vi "Acquisition.vi"(7 "CSM Name":string="CSM-Module") -> ()   [LabVIEW 2026, in "UI-温度控制.lvlib" / "Acquisition.lvlib"]
uses:
  Acquisition.lvlib
  Supports/Acquiring States.ctl
  Supports/Device Info.ctl
  Data ColndSave/Supports/Time and Data.ctl
  7c1bd55a-2ec8-456f-bad7-7e130b55c93f.vi
  2e6eb7ec-e133-45c6-ba3a-bbdf519762d0.vi
  817e4cca-a27d-44f6-a578-b7f1dff5f736.vi
  e4661991-72f6-45df-8df2-cd331cd0573d.vi
  d2ac0b8d-a34d-4c44-96e2-60a2cc9ef1dc.vi
  396d3fb3-9d86-4935-bc9b-05414301d3b2.vi
  e2432089-641f-414f-ac69-b6d04279e506.vi
  144ef8d5-f062-4612-a884-90947adc4c96.vi
  <userlib>/_NEVSTOP/Communicable State Machine(CSM)/AdvanceAPI/CSM - Revert Arguments-Safe String.vi
  <userlib>/_NEVSTOP/Communicable State Machine(CSM)/_Shared/Trim Single-line Text.vi
  <userlib>/_NEVSTOP/Communicable State Machine(CSM)/AdvanceAPI/CSM - Make String Arguments Safe.vi
  <userlib>/_NEVSTOP/Communicable State Machine(CSM)/AdvanceAPI/CSM - Break Down Multiple States String.vi
  <userlib>/_NEVSTOP/Communicable State Machine(CSM)/AdvanceAPI/CSM - Compact Multiple States.vi
  <userlib>/_NEVSTOP/Communicable State Machine(CSM)/AdvanceAPI/CSM - Keywords.vi
  <userlib>/_NEVSTOP/Communicable State Machine(CSM)/addons/API-String-Arugments-Support/_Support/Convert API String Arguments to Data(variant).vi
  <userlib>/_NEVSTOP/Communicable State Machine(CSM)/addons/MassData-Parameter/_support/FGV-MassData(lvlibp).vi
  <userlib>/_NEVSTOP/Communicable State Machine(CSM)/Communicable State Machine.lvlib
  <userlib>/_NEVSTOP/Communicable State Machine(CSM)/addons/Loop-Support/CSM Loop Support.lvlib
  Data ColndSave/Data Collection and Save.lvlib
panel:
  out "Error Occurred":errorcluster
  out "State History":string
  in  "Exit":bool
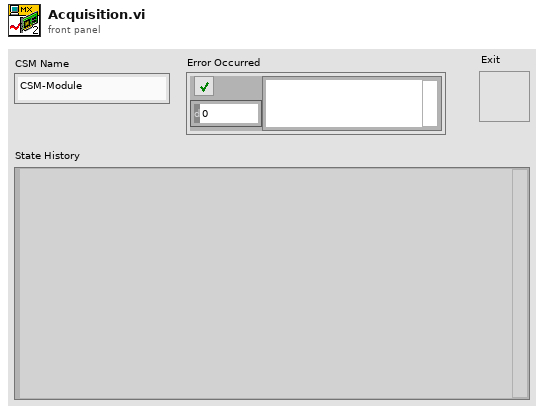
[diagram p1: front panel]
types:
  T1 = enum32{"Invalid", "Standard", "Closed", "Hidden", "Minimized", "Maximized"}
  T2 = enum32{"invalid app kind", "Development System", "Run Time System", "Student Edition", "Embedded LabVIEW", "Evaluation", "Custom"}
  T3 = typedef "UI-温度控制.lvlib/Acquisition.lvlib/Acquiring States.ctl" = enum16{"Idle", "Acquiring", "Error"}
  T4 = typedef "Data Collection and Save.lvlib/Time and Data.ctl" = cluster{"采集时间":timestamp, "Data":dbl[]}
  T5 = typedef "Communicable State Machine.lvlib/_CSM_Response Source Message.ctl" = cluster{"‘State":string, "’Arguments":string, "’Error":errorcluster}
  T6 = cluster{"Current VI Reference":refnum<vi>, "Close Panel on Exit?":bool}
  T7 = typedef "UI-温度控制.lvlib/Device Info.ctl" = cluster{"基本信息":cluster{"USB Port":refnum<visa-resource-name>, "采集间隔(s)":dbl}, "设备信息":cluster{"设备型号":string, "双通道设备？":bool}, "开关":cluster{"开关 1":bool, "开关 2":bool, "Fast Mode":bool}, "Control Temp":cluster{"Control Temp 1":dbl, "Control Temp 2":dbl}}
  T8 = cluster{"Core":cluster{"Current VI Reference":refnum<vi>, "Close Panel on Exit?":bool}, "State":T3, "Device Info":T7, "采集时间":timestamp}
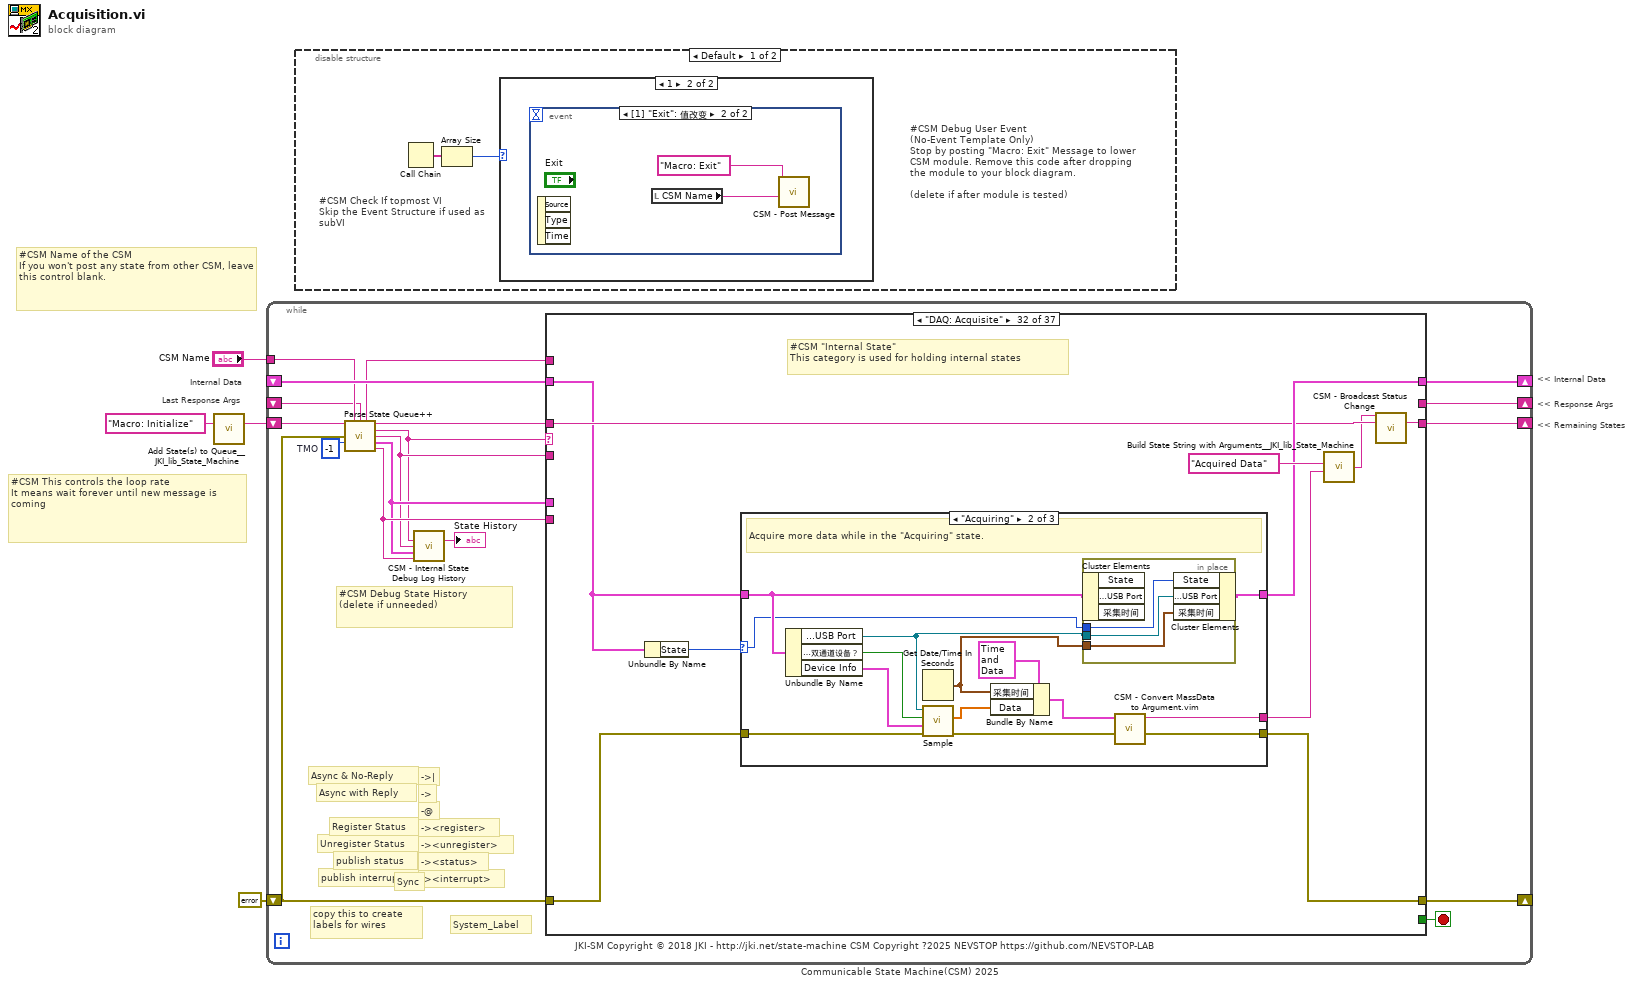
[diagram p0: block diagram]
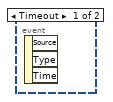
[diagram p3: hidden frame]
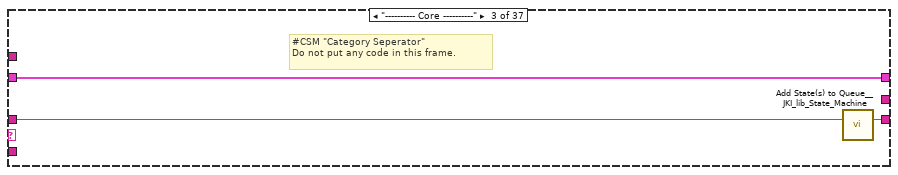
[diagram p7: hidden frame]
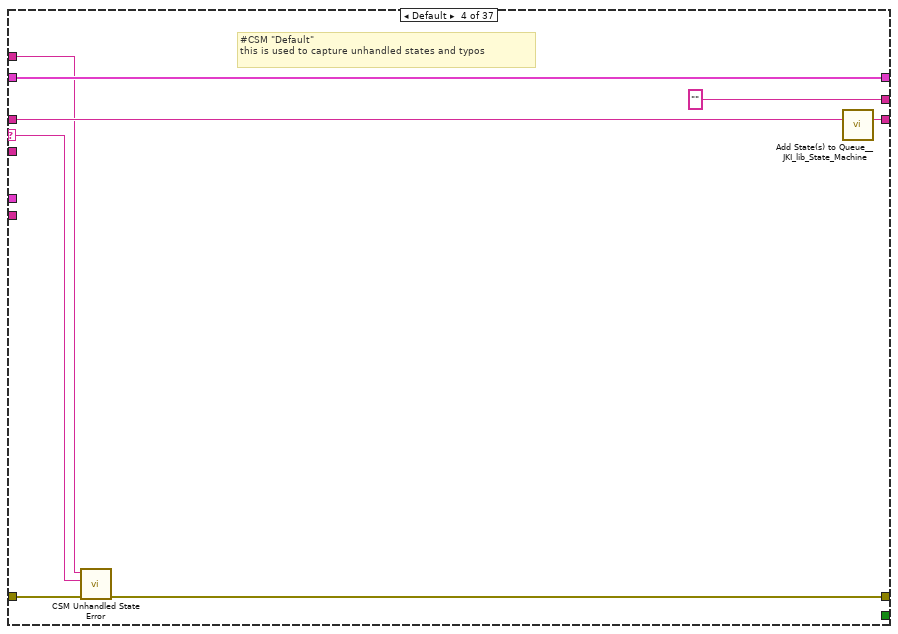
[diagram p8: hidden frame]
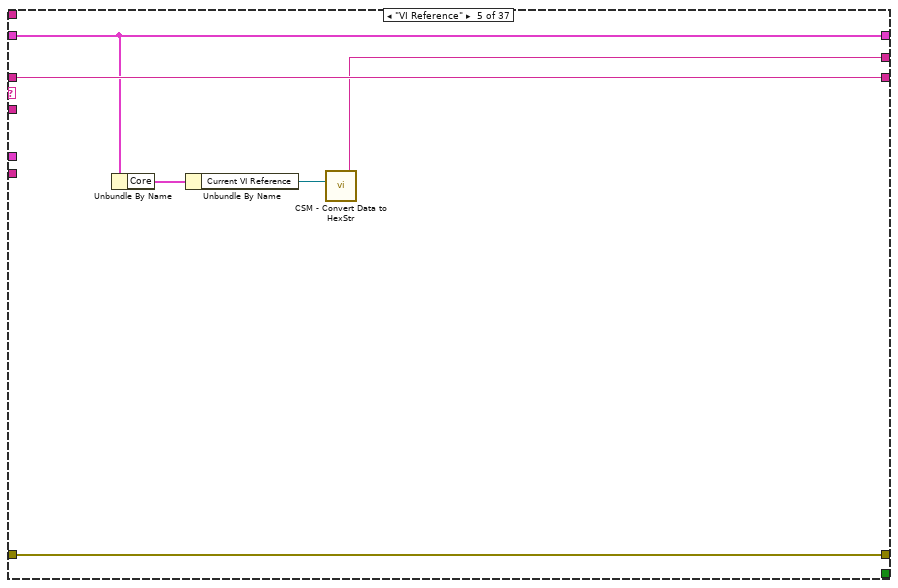
[diagram p9: hidden frame]
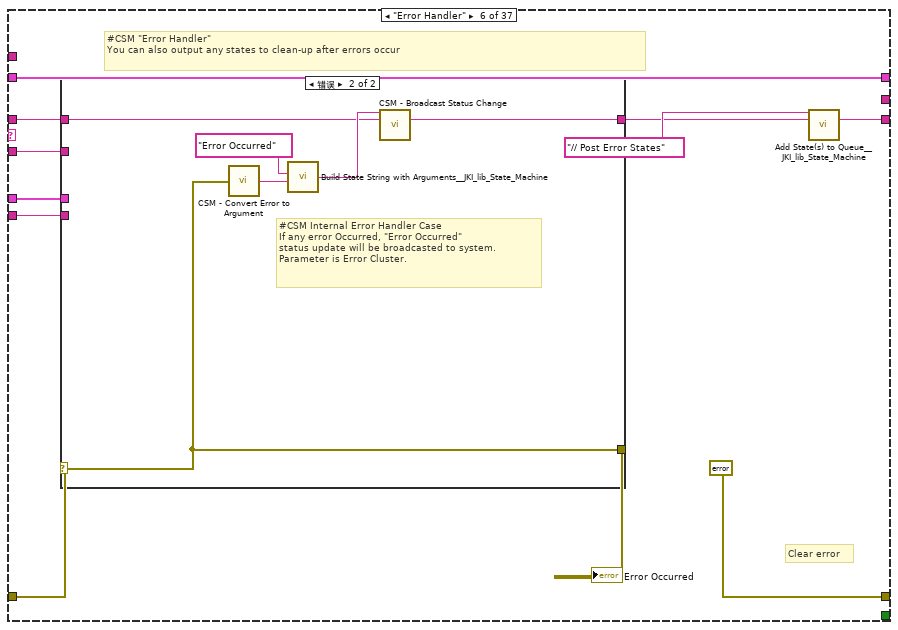
[diagram p10: hidden frame]
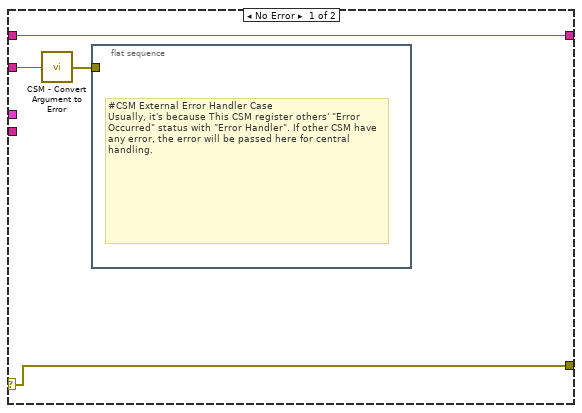
[diagram p11: hidden frame]
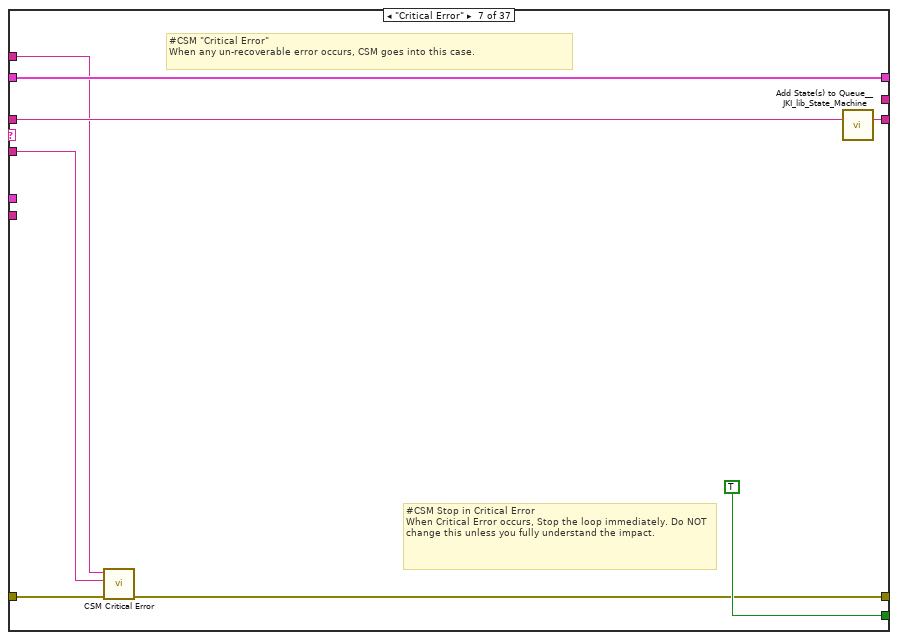
[diagram p12: hidden frame]
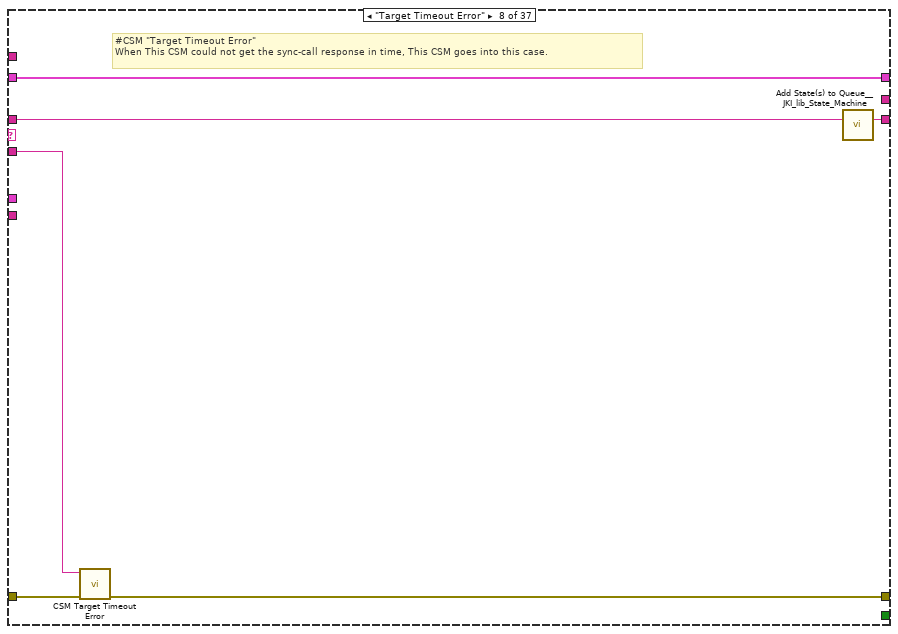
[diagram p13: hidden frame]
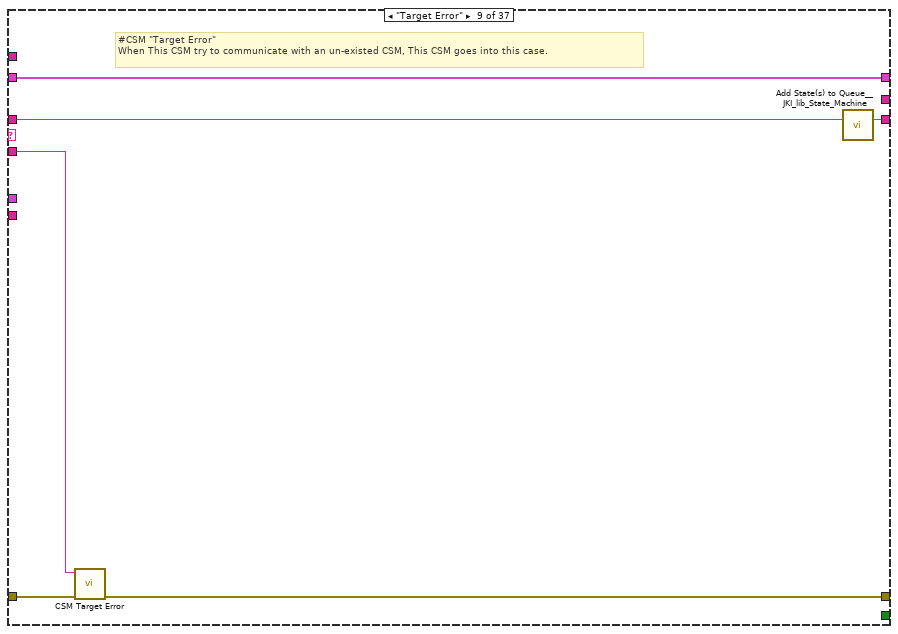
[diagram p14: hidden frame]
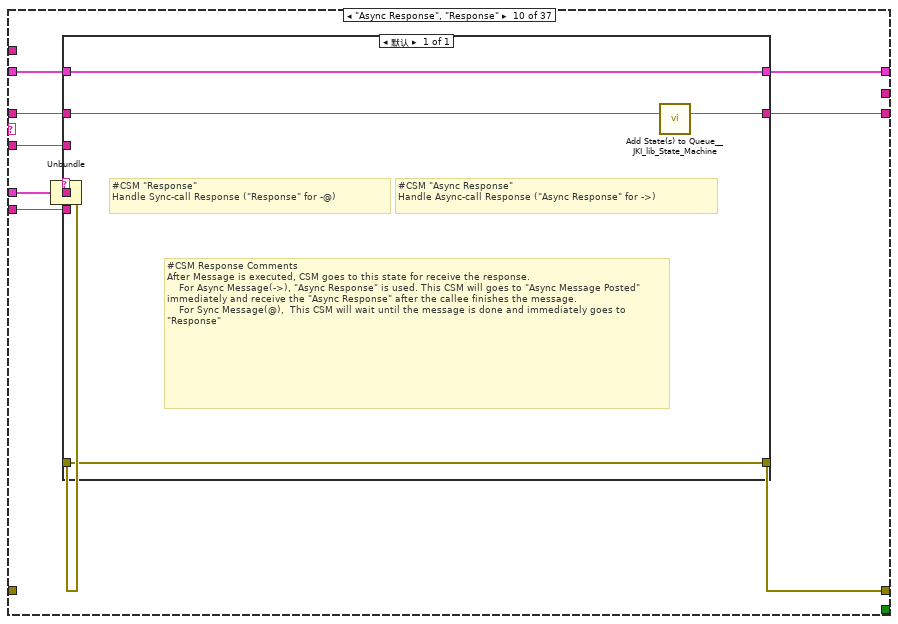
[diagram p15: hidden frame]
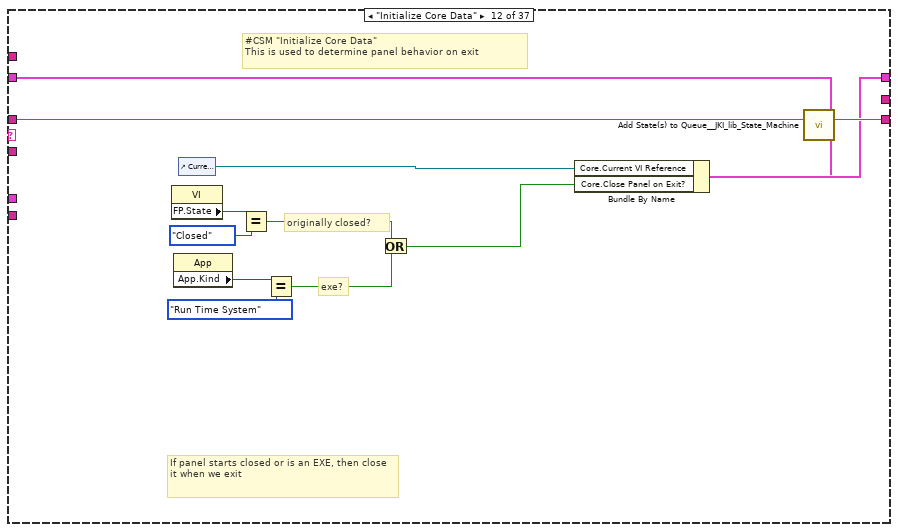
[diagram p17: hidden frame]
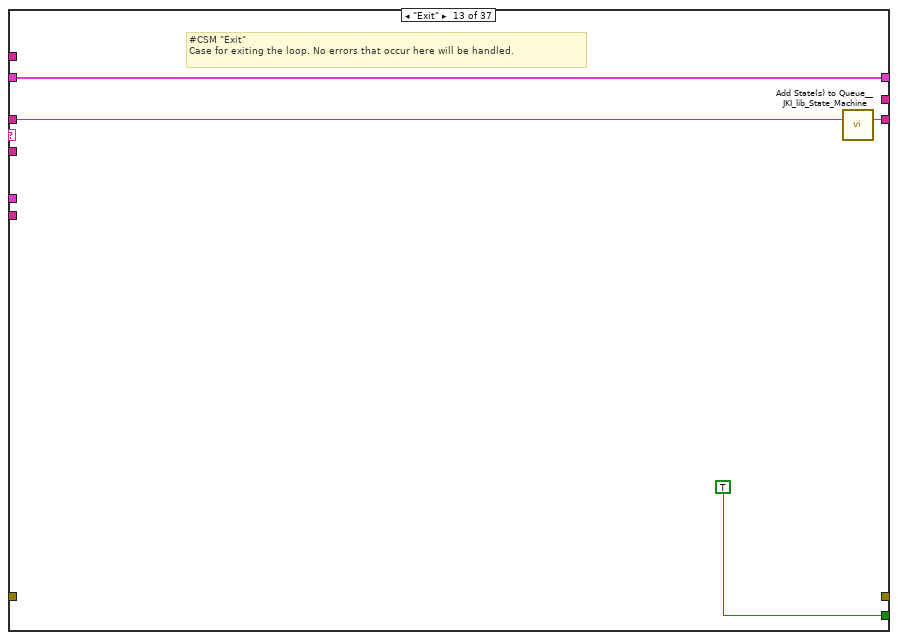
[diagram p18: hidden frame]
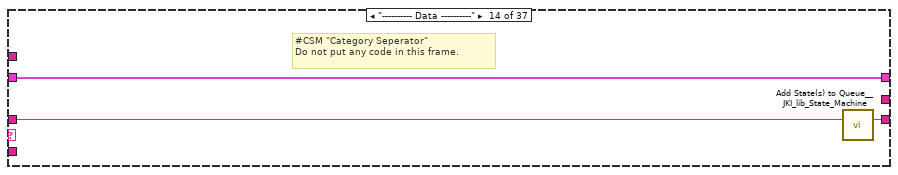
[diagram p19: hidden frame]
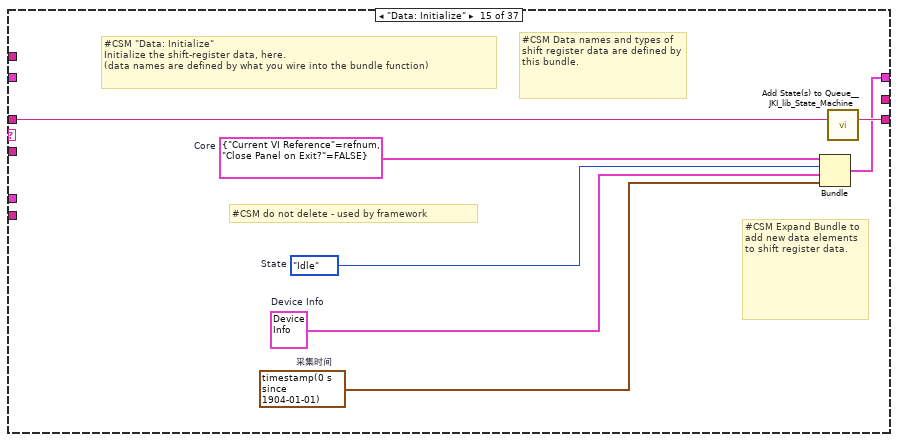
[diagram p20: hidden frame]
diagram:
  # "Last Response Args"
  # "Internal Data"
  # "#CSM Name of the CSM\nIf you won't post any state from other CSM, leave this control blank."
  # "#CSM This controls the loop rate\nIt means wait forever until new message is coming"
  # "<< Internal Data"
  # "<< Response Args"
  # "<< Remaining States"
  n1 = call <vilib>:"Add State(s) to Queue__JKI_lib_State_Machine.vi"("State(s) in (\"\")"="Macro: Initialize" ("Init State(\"Macro: Initialize\")")) -> ("States Out"=w1:string)  [unwired: 14 in]
  n2 = while "Communicable State Machine(CSM) 2025" {
    shift-right: [w17] -> _
    shift-left: _ -> [w16]
    shift-right: [w20] -> _
    shift-left: errorcluster {"status"=FALSE, "code"=0, "source"=""} ("error out") -> [w6]
    shift-right: [w19] -> _
    shift-left: w1 -> [w21]
    tunnel: "CSM Name" -> [w13]
    shift-right: [w14] -> _
    shift-left: _ -> [w8]
    stop <- w18 stop-if-true
    w15 = -1  # TMO
    # "#CSM Debug State History\n(delete if unneeded)"
    # "-><interrupt>"
    # "-><status>"
    # "-><unregister>"
    # "-><register>"
    # "-@"
    # "->"
    # "->|"
    # "publish interrupt"
    # "publish status"
    # "Unregister Status"
    # "Register Status"
    # "Sync"
    # "Async with Reply"
    # "Async & No-Reply"
    # "JKI-SM Copyright © 2018 JKI - http://jki.net/state-machine CSM Copyright ?2025 NEVSTOP https://github.com/NEVSTOP-LAB"
    # "copy this to create labels for wires"
    # "System_Label"
    n3 = call <userlib>:"Parse State Queue++.vi"("State Queue"=w21, "Name (\"\" to Use UUID)"=w13, "Response Arguments"=w8, "Previous Error"=w6, "Dequeue (1 ms)"=w15) -> ("Name Used"=w7:string, "Remaining States"=w22:string, "Current State"=w9:string, "Arguments"=w10:string, "Additional Information"=w11:T5, "Source CSM"=w12:string)  [unwired: 5 in]
    n4 = call <userlib>:"CSM - Internal State Debug Log History.vi"("State"=w9, "Arguments (\"\")"=w10, ">> Response Source Message >>"=w11, "Source (\"\")"=w12) -> ("Debug Log"=→"State History":string)  [unwired: 11 in]
    n5 = case shown="\"DAQ: Acquisite\"" w9 {
      selector: w9 -> [_ _ _ w33 _ _ _ _ _ _ _ _ _ _ _ _ _ _ _ _ _ _ _ _ _ _ _ _ _ _ _ _ _ _ _ w289 _]
      tunnel: w22 -> [w23 w26 w29 w37 w42 w48 w72 w78 w84 w94 w101 w113 w117 w120 w127 w130 w136 w139 w144 w153 w158 w163 w177 w182 w190 w198 w206 w215 w223 w232 w237 w241 w271 w276 w278 w291 w294]
      tunnel: w10 -> [_ _ _ _ _ w47 w68 w75 w81 w88 _ _ _ _ _ _ _ _ _ _ _ w160 _ w186 w194 w202 w210 w219 w227 _ _ _ _ _ _ w288 _]
      tunnel: w16 -> [w24 w25 w27 w35 w41 w53 w70 w76 w82 w92 w100 w107 w115 w118 _ w129 w131 w137 w142 w147 w157 w164 w179 w185 w193 w201 w209 w218 w226 w230 w234 w238 w269 w273 w277 w280 w295]
      tunnel: [_ _ _ w30 w43 errorcluster {"status"=FALSE, "code"=0, "source"=""} ("error out") w65 w73 w79 w95 _ _ _ _ _ _ w132 _ w140 w145 _ w159 w175 w189 w197 w205 w213 w221 w229 _ _ w243 _ _ w279 w292 w296] -> w20
      tunnel: w6 -> [_ _ _ w31 w43 w51 w66 w74 w80 _ _ _ _ _ _ _ w133 _ w140 w145 _ w159 w175 w189 w197 w205 w213 w221 w229 _ _ w242 _ _ w279 w292 w296]
      tunnel: [w23 w26 w28 w36 w42 w49 w71 w77 w83 w93 w101 w112 w116 w119 w126 w130 w135 w138 w143 w152 w158 w162 w178 w183 w191 w199 w207 w216 w224 w231 w236 w239 w270 w275 w278 w290 w293] -> w19
      tunnel: [_ _ _ _ _ _ TRUE _ _ _ _ _ TRUE _ _ _ _ _ _ _ _ _ _ _ _ _ _ _ _ _ _ _ _ _ _ _ _] -> w18
      tunnel: [w24 w25 w27 w35 w41 w53 w70 w76 w82 w91 w100 w111 w115 w118 w125 w129 w131 w137 w142 w147 w157 w161 w179 w184 w192 w200 w208 w217 w225 w230 w233 w244 w269 w272 w277 w280 w295] -> w17
      tunnel: w12 -> [_ _ _ _ _ w46 _ _ _ w89 _ _ _ _ _ _ _ _ _ _ _ _ _ _ _ _ _ _ _ _ _ _ _ _ _ _ _]
      tunnel: w11 -> [_ _ _ _ _ w45 _ _ _ w90 _ _ _ _ _ _ _ _ _ _ _ _ _ _ _ _ _ _ _ _ _ _ _ _ _ _ _]
      tunnel: [_ _ _ "" w38 _ _ _ _ _ _ _ _ _ _ _ _ _ _ _ _ _ _ _ _ _ _ _ _ _ _ _ _ _ _ _ _] -> w14
      tunnel: w7 -> [_ _ _ w32 _ _ w67 _ _ _ _ _ _ _ _ _ _ _ _ _ _ _ _ _ _ _ _ _ _ _ _ _ _ _ _ _ _]
      frame "", "Idle" {
        # "#CSM \"Idle/Event Handler\"\nexecutes when the state queue is empty"
      }
      frame "CSM Documentation" {
        # "#CSM State Syntax\n\n// Comment line, all text to the right of “//” will be ignored\n// Local Message Example\nDoSth: DoA >> Arguments\n\n// Sync Call Example\nAPI: xxxx >> Arguments -@ TargetModule\n\n// Async Call Example\nAPI: xxxx >> Arguments -> TargetModule\n\n// Async Call without Reply Example\nAPI: xxxx >> Arguments ->| TargetModule\n\n// Broadcast normal status:\nStatus >> StatusArguments  -><status>\n\n// Broadcast Interrupt status:\nInterrupt >> StatusArguments  -><interrupt>\n\n// Register Source Module's status to Handler Module\nStatus@Source Module >> Handler Module@Handler Module -><register>\n\n// Unegister Source Module's status\nStatus@Source Module >> Handler Module -><unregister>"
        # "#CSM README FIRST\n\nCommunicable State Machine(CSM) is a LabVIEW application framework that builds upon JKI State Machine(JKISM). It follows the pattern of JKISM and extends the keywords to describe message communication between modules, including concepts such as Sync-Message, Async-Message, Subscription/Unsubscription of status - essential elements for creating reusable code modules. For more information, please visit the CSM wiki: https://nevstop-lab.github.io/CSM-Wiki/\n\nFor instructions on JKI State Machine, visit: \n    http://jki.net/state-machine/\nFor information about CSM, visit: \n    https://github.com/NEVSTOP-LAB"
        # "#CSM \"Documentation\"\nCase for holding CSM Documenation"
      }
      frame "---------- Core ----------" {
        # "#CSM \"Category Seperator\"\nDo not put any code in this frame."
        n6 = call <vilib>:"Add State(s) to Queue__JKI_lib_State_Machine.vi"("State(s) in (\"\")"=w29) -> ("States Out"=w28:string)  [unwired: 14 in]
      }
      frame Default {
        # "#CSM \"Default\"\nthis is used to capture unhandled states and typos"
        n7 = call <userlib>:"CSM Unhandled State Error.vi"("error in (no error)"=w31, "Undefined State"=w33, "CSM Name"=w32) -> ("error out"=w30:errorcluster)  [unwired: 8 in]
        n8 = call <vilib>:"Add State(s) to Queue__JKI_lib_State_Machine.vi"("State(s) in (\"\")"=w37) -> ("States Out"=w36:string)  [unwired: 14 in]
      }
      frame "VI Reference" {
        n9 = Unbundle By Name(w41) -> ("Core"=w40:T6)
        n10 = Unbundle By Name(w40) -> ("Current VI Reference"=w39:refnum<vi>)
        n11 = call <userlib>:"CSM - Convert Data to HexStr.vi"("Variant"=w39) -> ("HEX String (0-9,A-F)"=w38:string)  [unwired: 8 in]
      }
      frame "Error Handler" {
        # "#CSM \"Error Handler\"\nYou can also output any states to clean-up after errors occur"
        # "Clear error"
        n12 = case shown="错误" w51 {
          selector: w51 -> [w55 w59]
          tunnel: [w58 w61] -> w50
          tunnel: w48 -> [w58 w60]
          tunnel: w47 -> [w57 _]
          tunnel: w46 -> [_ _]
          tunnel: w45 -> [_ _]
          tunnel: [w55 w59] -> w44
          frame No Error {
            n13 = call <userlib>:"CSM - Convert Argument to Error.vi"("Argument"=w57) -> ("Error"=w56:errorcluster)  [unwired: 4 in]
            n14 = flat-sequence {
              tunnel: w56 -> [_]
              frame #0 {
                # "#CSM External Error Handler Case\nUsually, it's because This CSM register others' \"Error Occurred\" status with \"Error Handler\". If other CSM have any error, the error will be passed here for central handling."
              }
            }
          }
          frame Error {
            # "#CSM Internal Error Handler Case \nIf any error Occurred, \"Error Occurred\" \nstatus update will be broadcasted to system.\nParameter is Error Cluster."
            n15 = call <userlib>:"CSM - Convert Error to Argument.vi"("Error"=w59) -> ("Argument"=w63:string)  [unwired: 4 in]
            n16 = call <vilib>:"Build State String with Arguments__JKI_lib_State_Machine.vi"("Arguments (\"\")"=w63, "State"="Error Occurred" ("Status with Arguments")) -> ("State with Arguments"=w62:string)  [unwired: 4 in]
            n17 = call <userlib>:"CSM - Broadcast Status Change.vi"("Status With Arguments"=w62, "State Queue"=w60) -> ("Remaining States"=w61:string)  [unwired: 13 in]
          }
        }
        "Error Occurred" <- w44
        n18 = call <vilib>:"Add State(s) to Queue__JKI_lib_State_Machine.vi"("State(s) in Front (\"\")"="// Post Error States", "State(s) in (\"\")"=w50) -> ("States Out"=w49:string)  [unwired: 13 in]
      }
      frame "Critical Error" {
        # "#CSM \"Critical Error\"\nWhen any un-recoverable error occurs, CSM goes into this case."
        # "#CSM Stop in Critical Error\nWhen Critical Error occurs, Stop the loop immediately. Do NOT change this unless you fully understand the impact."
        n19 = call <userlib>:"CSM Critical Error.vi"("error in (no error)"=w66, "Arugments (As Reason)"=w68, "CSM Name"=w67) -> ("error out"=w65:errorcluster)  [unwired: 8 in]
        n20 = call <vilib>:"Add State(s) to Queue__JKI_lib_State_Machine.vi"("State(s) in (\"\")"=w72) -> ("States Out"=w71:string)  [unwired: 14 in]
      }
      frame "Target Timeout Error" {
        # "#CSM \"Target Timeout Error\"\nWhen This CSM could not get the sync-call response in time, This CSM goes into this case."
        n21 = call <userlib>:"CSM Target Timeout Error.vi"("error in (no error)"=w74, "Arguments (As CSM Name)"=w75) -> ("error out"=w73:errorcluster)  [unwired: 9 in]
        n22 = call <vilib>:"Add State(s) to Queue__JKI_lib_State_Machine.vi"("State(s) in (\"\")"=w78) -> ("States Out"=w77:string)  [unwired: 14 in]
      }
      frame "Target Error" {
        # "#CSM \"Target Error\"\nWhen This CSM try to communicate with an un-existed CSM, This CSM goes into this case."
        n23 = call <userlib>:"CSM Target Error.vi"("error in (no error)"=w80, "Arguments (As CSM Name)"=w81) -> ("error out"=w79:errorcluster)  [unwired: 9 in]
        n24 = call <vilib>:"Add State(s) to Queue__JKI_lib_State_Machine.vi"("State(s) in (\"\")"=w84) -> ("States Out"=w83:string)  [unwired: 14 in]
      }
      frame "Async Response", "Response" {
        n25 = Unbundle(w90) -> ("‘State"=w87:string, "’Arguments"=w86:string, "’Error"=w85:errorcluster)
        n26 = case shown="默认" w87 {
          tunnel: [w96] -> w93
          tunnel: w94 -> [w97]
          tunnel: [w99] -> w91
          tunnel: w92 -> [w99]
          tunnel: [w98] -> w95
          tunnel: w85 -> [w98]
          tunnel: w89 -> [_]
          tunnel: w88 -> [_]
          tunnel: w86 -> [_]
          frame 默认 {
            # "#CSM \"Async Response\"\nHandle Async-call Response (\"Async Response\" for ->)"
            # "#CSM \"Response\"\nHandle Sync-call Response (\"Response\" for -@)"
            # "#CSM Response Comments\nAfter Message is executed, CSM goes to this state for receive the response.\n    For Async Message(->), \"Async Response\" is used. This CSM will goes to \"Async Message Posted\" immediately and receive the \"Async Response\" after the callee finishes the message.\n    For Sync Message(@),  This CSM will wait until the message is done and immediately goes to \"Response\""
            n27 = call <vilib>:"Add State(s) to Queue__JKI_lib_State_Machine.vi"("State(s) in (\"\")"=w97) -> ("States Out"=w96:string)  [unwired: 14 in]
          }
        }
      }
      frame "Async Message Posted" {
        # "#CSM \"Async Message Posted\"\nAfter Async Message is posted (-> or ->| ), CSM goes to this state for post-action.\nYou can use Argument - State to tell which Async Message is called."
      }
      frame "Initialize Core Data" {
        # "#CSM \"Initialize Core Data\"\nThis is used to determine panel behavior on exit"
        # "originally closed?"
        # "exe?"
        # "If panel starts closed or is an EXE, then close it when we exit"
        n28 = property class="VI"() -> ("FP.State"=w104:T1)  [unwired: 2 in, 2 out]
        n29 = property class="App"() -> ("App.Kind"=w110:T2)  [unwired: 2 in, 2 out]
        n30 = control-ref of="Current VI Reference"() -> (w105:refnum<vi>)
        n31 = Equal?(x=w104, y=T1."Closed" ("Front Panel Window:State")) -> (x = y?=w102:bool)
        n32 = Equal?(x=w110, y=T2."Run Time System" ("Application:Kind")) -> (x = y?=w108:bool)
        n33 = Or(x=w102, y=w108) -> (x .or. y?=w106:bool)
        n34 = Bundle By Name(cluster=w107, "Core.Current VI Reference"=w105, "Core.Close Panel on Exit?"=w106) -> (w111:T8)
        n35 = call <vilib>:"Add State(s) to Queue__JKI_lib_State_Machine.vi"("State(s) in (\"\")"=w113) -> ("States Out"=w112:string)  [unwired: 14 in]
      }
      frame "Exit" {
        # "#CSM \"Exit\"\nCase for exiting the loop. No errors that occur here will be handled."
        n36 = call <vilib>:"Add State(s) to Queue__JKI_lib_State_Machine.vi"("State(s) in (\"\")"=w117) -> ("States Out"=w116:string)  [unwired: 14 in]
      }
      frame "---------- Data ----------" {
        # "#CSM \"Category Seperator\"\nDo not put any code in this frame."
        n37 = call <vilib>:"Add State(s) to Queue__JKI_lib_State_Machine.vi"("State(s) in (\"\")"=w120) -> ("States Out"=w119:string)  [unwired: 14 in]
      }
      frame "Data: Initialize" {
        w121 = timestamp(0 s since 1904-01-01)  # 采集时间
        w122 = T7 {"基本信息"={"USB Port"="", "采集间隔(s)"=0.0}, "设备信息"={"设备型号"="", "双通道设备？"=FALSE}, "开关"={"开关 1"=FALSE, "开关 2"=FALSE, "Fast Mode"=FALSE}, "Control Temp"={"Control Temp 1"=0.0, "Control Temp 2"=0.0}}  # Device Info
        w123 = Acquiring_States."Idle"  # State
        w124 = T6 {"Current VI Reference"=refnum, "Close Panel on Exit?"=FALSE}  # Core
        # "#CSM \"Data: Initialize\"\nInitialize the shift-register data, here.\n(data names are defined by what you wire into the bundle function)"
        # "#CSM do not delete - used by framework"
        # "#CSM Expand Bundle to add new data elements to shift register data."
        # "#CSM Data names and types of shift register data are defined by this bundle."
        n38 = Bundle("Core"=w124, "State"=w123, "Device Info"=w122, "采集时间"=w121) -> (w125:T8)  [unwired: 1 in]
        n39 = call <vilib>:"Add State(s) to Queue__JKI_lib_State_Machine.vi"("State(s) in (\"\")"=w127) -> ("States Out"=w126:string)  [unwired: 14 in]
      }
      frame "Data: Update Indicators" {
        n40 = local write "Error Occurred"(errorcluster {"status"=FALSE, "code"=0, "source"=""} ("错误常量")) -> ()
      }
      frame "Data: Cleanup" {
        # "#CSM \"Data: Cleanup\"\nCleanup any data and references, here.\n(this is called automatically, by the Macro: Exit)"
        n41 = Unbundle By Name(w131) -> ("Core.Current VI Reference"=w134:refnum<vi>)
        n42 = Close Reference(reference=w134, error in (no error)=w133) -> (error out=w132:errorcluster)
        n43 = call <vilib>:"Add State(s) to Queue__JKI_lib_State_Machine.vi"("State(s) in (\"\")"=w136) -> ("States Out"=w135:string)  [unwired: 14 in]
      }
      frame "---------- Macro ----------" {
        # "#CSM \"Category Seperator\"\nDo not put any code in this frame."
        n44 = call <vilib>:"Add State(s) to Queue__JKI_lib_State_Machine.vi"("State(s) in (\"\")"=w139) -> ("States Out"=w138:string)  [unwired: 14 in]
      }
      frame "Macro: Initialize" {
        # "#CSM \"Macro: Initialize\"\nInitialization Macro (This is called once, when the VI starts)"
        n45 = call <vilib>:"Add State(s) to Queue__JKI_lib_State_Machine.vi"("State(s) in Front (\"\")"="Data: Initialize\nInitialize Core Data\nData: Update Indicators", "State(s) in (\"\")"=w144) -> ("States Out"=w143:string)  [unwired: 13 in]
      }
      frame "Macro: Exit" {
        # "#CSM \"Macro: Exit\"\nExit Macro (This is called once, when the VI exits)"
        n46 = Unbundle By Name(w147) -> ("State"=w148:T3)
        n47 = case shown="\"Acquiring\"" w148 {
          tunnel: ["" "Break Continuous" ""] -> w146
          frame "Idle", Default {
          }
          frame "Acquiring" {
          }
          frame "Error" {
          }
        }
        n48 = call <vilib>:"Add State(s) to Queue__JKI_lib_State_Machine.vi"("State(s) in Front (\"\")"="//Exit Sub-Modules ", "State(s) in (\"\")"=w146, "State(s) at Back (\"\")"="Data: Cleanup\nExit") -> ("States Out"=w150:string)  [unwired: 12 in]
        n49 = call <vilib>:"Add State(s) to Queue__JKI_lib_State_Machine.vi"("State(s) in Front (\"\")"=w150, "State(s) in (\"\")"=w153) -> ("States Out"=w152:string)  [unwired: 13 in]
      }
      frame "---------- API ----------" {
        # "#CSM \"Category Seperator\"\nDo not put any code in this frame."
      }
      frame "API: Start" {
        # "#CSM API Example\nCopy/Rename this case for your own API"
        # "#CSM API Example\nCopy/Rename this case for your own API"
        n50 = Unbundle By Name(w164) -> ("State"=w167:T3)
        n51 = Unbundle By Name(w164) -> ("Device Info"=w170:T7)
        n52 = case shown="\"Idle\"" w167 {
          selector: w167 -> [_ w173 w174]
          tunnel: [Acquiring_States."Acquiring" ("Acquisition State") w173 w174] -> w166
          tunnel: ["DAQ: Initialize \nDAQ: Acquisite\nContinuous Check >> DAQ: Acquisite -><loop> \nDAQ: Close " ("State(s) in Front (\"\")") _ _] -> w168
          frame "Idle" {
            # "If the system is idle, start the acquisition."
          }
          frame "Acquiring" {
            # "The system is already acquiring. Ignore the \"Start\" message."
          }
          frame "Error" {
          }
        }
        n53 = local write "Error Occurred"(errorcluster {"status"=FALSE, "code"=0, "source"=""} ("错误常量")) -> ()
        n54 = call "Convert API String Arguments to Data.vim"("Reference Type"=w170, "API String"=w160) -> ("Data"=w169:T7)  [unwired: 6 in, 1 out]
        n55 = call <userlib>:"CSMLS - Define Loop State(s).vi"("Loop States"=w168, "States Queue"=w163) -> ("Remaining States"=w162:string)  [unwired: 13 in]
        n56 = Bundle By Name(cluster=w164, "State"=w166, "Device Info"=w169) -> (w161:T8)
      }
      frame "API: Stop" {
        # "#CSM API Example\nCopy/Rename this case for your own API"
        n57 = Unbundle By Name(w179) -> ("State"=w180:T3)
        n58 = case shown="\"Acquiring\"" w180 {
          tunnel: [_ "Break Continuous" ("State(s) in Front (\"\")") _] -> w176
          frame "Idle" {
            # "The system is already idle. Ignore the \"Stop\" message."
          }
          frame "Acquiring" {
            # "If the system is acquiring, stop the acquisition."
          }
          frame "Error" {
          }
        }
        n59 = call <vilib>:"Add State(s) to Queue__jki_lib_state_machine.vi"("State(s) in Front (\"\")"=w176, "State(s) in (\"\")"=w177) -> ("States Out"=w178:string)  [unwired: 13 in]
      }
      frame "API: ONOFF1" {
        n60 = call "Convert API String Arguments to Data.vim"("Reference Type"=FALSE, "API String"=w186) -> ("Data"=w187:bool)  [unwired: 6 in, 1 out]
        n61 = Bundle By Name(cluster=w185, "Device Info.开关.开关 1"=w187) -> (w184:T8)
        n62 = call <vilib>:"Add State(s) to Queue__jki_lib_state_machine.vi"("State(s) in (\"\")"=w182) -> ("States Out"=w183:string)  [unwired: 14 in]
      }
      frame "API: ONOFF2" {
        n63 = call "Convert API String Arguments to Data.vim"("Reference Type"=FALSE, "API String"=w194) -> ("Data"=w195:bool)  [unwired: 6 in, 1 out]
        n64 = Bundle By Name(cluster=w193, "Device Info.开关.开关 2"=w195) -> (w192:T8)
        n65 = call <vilib>:"Add State(s) to Queue__jki_lib_state_machine.vi"("State(s) in (\"\")"=w190) -> ("States Out"=w191:string)  [unwired: 14 in]
      }
      frame "API: Fast Mode" {
        n66 = call "Convert API String Arguments to Data.vim"("Reference Type"=FALSE, "API String"=w202) -> ("Data"=w203:bool)  [unwired: 6 in, 1 out]
        n67 = Bundle By Name(cluster=w201, "Device Info.开关.Fast Mode"=w203) -> (w200:T8)
        n68 = call <vilib>:"Add State(s) to Queue__jki_lib_state_machine.vi"("State(s) in (\"\")"=w198) -> ("States Out"=w199:string)  [unwired: 14 in]
      }
      frame "API: Sample Interval" {
        n69 = call "Convert API String Arguments to Data.vim"("Reference Type"=0.0, "API String"=w210) -> ("Data"=w211:dbl)  [unwired: 6 in, 1 out]
        n70 = Bundle By Name(cluster=w209, "Device Info.基本信息.采集间隔(s)"=w211) -> (w208:T8)
        n71 = call <vilib>:"Add State(s) to Queue__jki_lib_state_machine.vi"("State(s) in (\"\")"=w206) -> ("States Out"=w207:string)  [unwired: 14 in]
      }
      frame "API: Control Temp 1" {
        n72 = call "Convert API String Arguments to Data.vim"("Reference Type"=0.0, "API String"=w219) -> ("Data"=w214:dbl)  [unwired: 6 in, 1 out]
        n73 = Bundle By Name(cluster=w218, "Device Info.Control Temp.Control Temp 1"=w214) -> (w217:T8)
        n74 = call <vilib>:"Add State(s) to Queue__jki_lib_state_machine.vi"("State(s) in (\"\")"=w215) -> ("States Out"=w216:string)  [unwired: 14 in]
      }
      frame "API: Control Temp 12 " {
        n75 = call "Convert API String Arguments to Data.vim"("Reference Type"=0.0, "API String"=w227) -> ("Data"=w222:dbl)  [unwired: 6 in, 1 out]
        n76 = Bundle By Name(cluster=w226, "Device Info.Control Temp.Control Temp 2"=w222) -> (w225:T8)
        n77 = call <vilib>:"Add State(s) to Queue__jki_lib_state_machine.vi"("State(s) in (\"\")"=w223) -> ("States Out"=w224:string)  [unwired: 14 in]
      }
      frame "---------- DAQ ----------" {
        # "#CSM \"Category Seperator\"\nDo not put any code in this frame."
        n78 = call <vilib>:"Add State(s) to Queue__JKI_lib_State_Machine.vi"("State(s) in (\"\")"=w232) -> ("States Out"=w231:string)  [unwired: 14 in]
      }
      frame "DAQ: Initialize" {
        # "#CSM \"Category Seperator\"\nDo not put any code in this frame."
        n79 = Unbundle By Name(w234) -> ("Device Info.基本信息.USB Port"=w235:refnum<visa-resource-name>)
        n80 = Bundle By Name(cluster=w234, "Device Info.基本信息.USB Port"=w235) -> (w233:T8)
        n81 = call <vilib>:"Add State(s) to Queue__JKI_lib_State_Machine.vi"("State(s) in (\"\")"=w237) -> ("States Out"=w236:string)  [unwired: 14 in]
      }
      frame "DAQ: Acquisite" {
        # "#CSM \"Internal State\"\nThis category is used for holding internal states"
        n82 = Unbundle By Name(w238) -> ("State"=w247:T3)
        n83 = case shown="\"Acquiring\"" w247 {
          selector: w247 -> [_ w252 _]
          tunnel: [w249 w262 w268] -> w243
          tunnel: w242 -> [w249 w261 w268]
          tunnel: [w248 w253 w267] -> w244
          tunnel: w238 -> [w248 w254 w267]
          tunnel: [_ w263 _] -> w245
          frame "Idle" {
            # "Ignore \"Acquire\" messages when the acquisition is idle."
          }
          frame "Acquiring" {
            # "Acquire more data while in the \"Acquiring\" state."
            n84 = Unbundle By Name(w254) -> ("Device Info.基本信息.USB Port"=w251:refnum<visa-resource-name>, "Device Info.设备信息.双通道设备？"=w257:bool, "Device Info"=w255:T7)
            n85 = Get Date/Time In Seconds() -> (seconds since 1Jan1904=w250:timestamp)
            n86 = call "Sample.vi"("错误输入（无错误）"=w261, "Device Info.开关"=w255, "双通道设备？"=w257, "VISA资源名称"=w251) -> ("error out"=w260:errorcluster, "Data Out"=w256:dbl[])  [unwired: 6 in]
            n87 = Bundle By Name(cluster=T4 {"采集时间"=timestamp(0 s since 1904-01-01), "Data"=[]} ("Time and Data"), "采集时间"=w250, "Data"=w256) -> (w258:T4)
            n88 = in-place {
              in-place-border: w252 -> [w266]
              in-place-border: w251 -> [w264]
              in-place-border: w250 -> [w265]
              n89 = in-place-cluster #1(w254) -> ()  [unwired: 3 out]
              n90 = in-place-cluster #1("State"=w266, "Device Info.基本信息.USB Port"=w264, "采集时间"=w265) -> (w253:T8)
            }
            n91 = call "CSM - Convert MassData to Argument.vim"("error in (no error)"=w260, "Data"=w258) -> ("error out"=w262:errorcluster, "MassData Argument"=w263:string)  [unwired: 6 in]
          }
          frame "Error" {
          }
        }
        n92 = call <vilib>:"Build State String with Arguments__JKI_lib_State_Machine.vi"("Arguments (\"\")"=w245, "State"="Acquired Data" ("Status with Arguments")) -> ("State with Arguments"=w240:string)  [unwired: 4 in]
        n93 = call <userlib>:"CSM - Broadcast Status Change.vi"("Status With Arguments"=w240, "State Queue"=w241) -> ("Remaining States"=w239:string)  [unwired: 13 in]
      }
      frame "DAQ: Stop" {
        # "#CSM \"Internal State\"\nThis category is used for holding internal states"
        n94 = call <vilib>:"Add State(s) to Queue__JKI_lib_State_Machine.vi"("State(s) in (\"\")"=w271) -> ("States Out"=w270:string)  [unwired: 14 in]
      }
      frame "DAQ: Close" {
        w274 = Acquiring_States."Idle"  # State
        # "#CSM \"Internal State\"\nThis category is used for holding internal states"
        n95 = Bundle By Name(cluster=w273, "State"=w274) -> (w272:T8)
        n96 = call <vilib>:"Add State(s) to Queue__JKI_lib_State_Machine.vi"("State(s) in (\"\")"=w276) -> ("States Out"=w275:string)  [unwired: 14 in]
      }
      frame "---------- Loop ----------" {
      }
      frame "Continuous Check" {
        n97 = Unbundle By Name(w280) -> ("Device Info.基本信息.采集间隔(s)"=w287:dbl, "采集时间"=w284:timestamp)
        n98 = Get Date/Time In Seconds() -> (seconds since 1Jan1904=w285:timestamp)
        n99 = Multiply(x=u32 1000 ("y"), y=w287) -> (x*y=w283:dbl)
        n100 = Subtract(x=w285, y=w284) -> (x-y=w282:dbl)
        n101 = Subtract(x=w283, y=w282) -> (x-y=w281:dbl)
        n102 = Wait (ms)(milliseconds to wait=w281) -> ()  [unwired: 1 out]
        n103 = call <userlib>:"CSMLS - Append Continuous State.vi"("Loop State(s) And Arguments"=w288, "Continous Arguments (\"\")"=w288, "Continous State"=w289, "States Queue"=w291) -> ("Remaining States"=w290:string)  [unwired: 7 in]
      }
      frame "Break Continuous" {
        n104 = call <userlib>:"CSMLS - Remove Loop Tag to Break.vi"("States Queue"=w294) -> ("Remaining States"=w293:string)  [unwired: 10 in]
      }
    }
  }
  n105 = disable-structure shown="Default" {
    frame condition #0 (active) {
      # "#CSM Check If topmost VI\nSkip the Event Structure if used as subVI"
      # "#CSM Debug User Event\n(No-Event Template Only)\nStop by posting \"Macro: Exit\" Message to lower CSM module. Remove this code after dropping the module to your block diagram. \n\n(delete if after module is tested)"
      n106 = Call Chain() -> (call chain=w298:string[])
      n107 = Array Size(array=w298) -> (size(s)=w297:i32)
      n108 = case shown="1" w297 {
        frame Default {
        }
        frame 1 {
          n109 = event shown="[1] \"Exit\": 值改变" {
            selector: _ -> [_ _]
            dyn-events: _ -> [_ _]
            timeout: _ -> [_ _]
            event Timeout {
              n110 = event-data() -> ()  [unwired: 1 in, 3 out]
            }
            event "Exit": Value Change {
              n111 = event-data() -> ()  [unwired: 1 in, 3 out]
              n112 = local read "CSM Name"() -> (w300:string)
              n113 = call <userlib>:"CSM - Post Message.vi"("Target Module"=w300, "State"="Macro: Exit" ("States")) -> ()  [unwired: 9 in, 1 out]
            }
          }
        }
      }
    }
    frame condition #1 {
    }
  }
